vi "WaitOn_Queue.vi"(5 "Blackboard Group":string="Default", 6 "Tag Root":string, 7 "Queue Name":string, 8 "Max Queue Size":i32=-1, 9 "Timeout (ms)":i32=-1, 10 "Message Type":variant, 11 "bt_Blackboard in":refnum<class "Blackboard.lvclass">) -> (0 "error out":errorcluster, 3 "Node Out":refnum<class "bt_Node.lvclass">)   [LabVIEW 2021, in "BT.lvlib"]
uses:
  Blackboard/Blackboard.lvclass
  Support/Nodes/Leaves/Synch/Queue/WaitOn/bt_WaitOn_Queue.lvclass/bt_WaitOn_Queue.ctl
  Support/Nodes/Leaves/Synch/Parent/WaitOn/bt_WaitOn_Synch.lvclass/bt_WaitOn_Synch.ctl
  Support/Nodes/Leaves/Synch/Queue/WaitOn/Properties/Write Name.vi
  Support/Nodes/Leaves/Synch/Queue/WaitOn/Properties/Write Max Queue Size.vi
  Support/Nodes/Leaves/Synch/Parent/WaitOn/Properties/Write Timeout.vi
  Support/Nodes/Leaves/Synch/Queue/WaitOn/Properties/Write bt_Blackboard.vi
  Support/Nodes/Leaves/Synch/Queue/WaitOn/Properties/Write Message Type.vi
  Support/Nodes/Leaves/Synch/Queue/WaitOn/Properties/Write Tag Root.vi
  Support/Nodes/Leaves/Synch/Queue/WaitOn/Properties/Write Blackboard Group.vi
  BT.lvlib
  Support/Nodes/Leaves/Synch/Queue/WaitOn/bt_WaitOn_Queue.lvclass
  C:/Users/Tim/Documents/GitHub/LV_Behaviour_Tree/Source/Support/Nodes/Leaves/Synch/With Values/WaitOn/bt_WaitOn_Synch_WithValues.lvclass
  C:/Users/Tim/Documents/GitHub/LV_Behaviour_Tree/Source/Support/Nodes/Leaves/Synch/Parent/WaitOn/bt_WaitOn_Synch.lvclass
  C:/Users/Tim/Documents/GitHub/LV_Behaviour_Tree/Source/Support/Nodes/Leaves/Leaf/bt_Leaf.lvclass
  C:/Users/Tim/Documents/GitHub/LV_Behaviour_Tree/Source/Support/Nodes/abs_Node/bt_Node.lvclass
  C:/Users/Tim/Documents/GitHub/LV_Behaviour_Tree/Source/Support/Nodes/Leaves/Synch/Queue/WaitOn/bt_WaitOn_Queue.lvclass
  Support/Nodes/abs_Node/bt_Node.lvclass
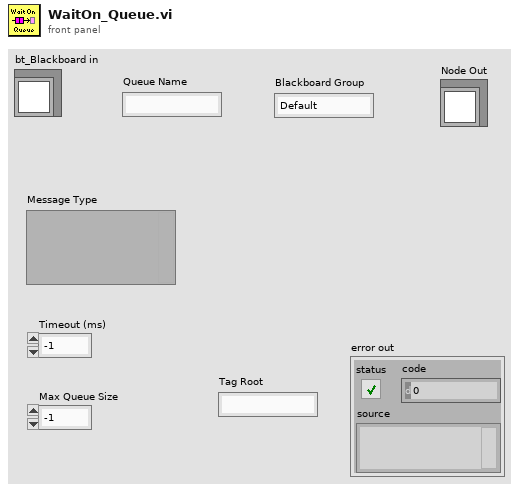
[diagram p1: front panel]
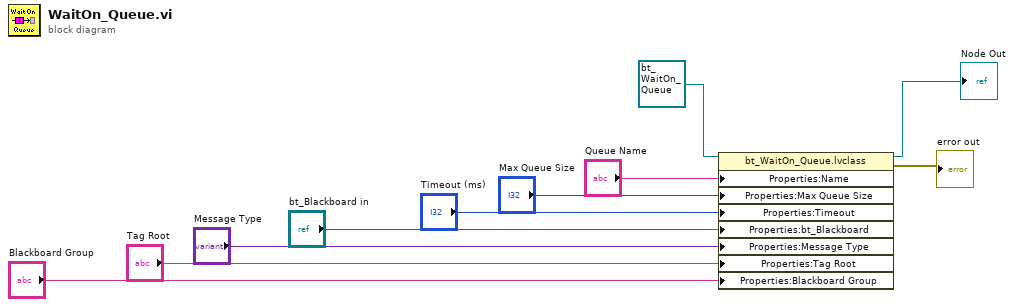
[diagram p0: block diagram]
diagram:
  n1 = property class="bt_WaitOn_Queue.lvclass"(reference=refnum<class "bt_WaitOn_Queue.lvclass"> refnum ("BT.lvlib:bt_WaitOn_Queue.lvclass"), "Properties:Name"="Queue Name", "Properties:Max Queue Size"="Max Queue Size", "Properties:Timeout"="Timeout (ms)", "Properties:bt_Blackboard"="bt_Blackboard in", "Properties:Message Type"="Message Type", "Properties:Tag Root"="Tag Root", "Properties:Blackboard Group"="Blackboard Group") -> (reference out=→"Node Out":refnum<class "bt_WaitOn_Queue.lvclass">, error out=→"error out":errorcluster)  [unwired: 1 in]
